vi "Routes.vi"() -> (3 "Routes":T1[](array[typedef]))   [LabVIEW 2024]
doc: "Configure routes"
uses:
  NavigatableView/NavigatableView.lvclass
  Navigator/Route.ctl
  Navigator/Navigator.lvclass
  Pages/Page1/View/View.lvclass
  Pages/Page2/View/View.lvclass
  C:/Users/N Tan/Documents/1-Reuse Modules/Navigator/NavigatableView/NavigatableView.lvclass
  C:/Users/N Tan/Documents/1-Reuse Modules/Navigator/Example/Pages/Page1/View/View.lvclass
  C:/Users/N Tan/Documents/1-Reuse Modules/Navigator/Example/Pages/Page2/View/View.lvclass
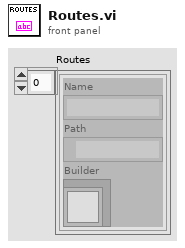
[diagram p1: front panel]
types:
  T1 = typedef "Navigator.lvclass/Route.ctl" = cluster{"Name":string, "Path":path, "Builder":refnum<class "NavigatableView.lvclass">}
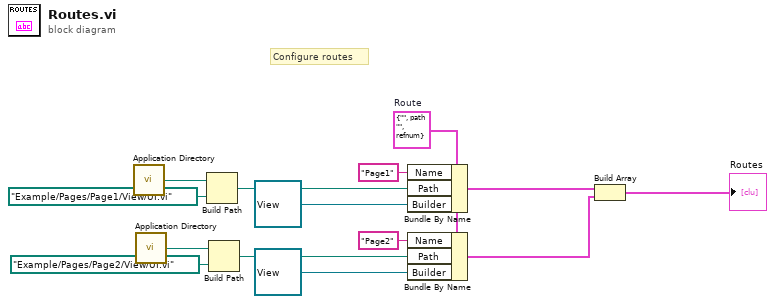
[diagram p0: block diagram]
diagram:
  w10 = T1 {"Name"="", "Path"=path "", "Builder"=refnum}  # Route
  # "Configure routes"
  n1 = call <vilib>:"Application Directory.vi"() -> ("Application Directory"=w8:path)
  n2 = call <vilib>:"Application Directory.vi"() -> ("Application Directory"=w4:path)
  n3 = Build Path(base path=w8, name or relative path=path "Example/Pages/Page1/View/UI.vi") -> (appended path=w6:path)
  n4 = Build Path(base path=w4, name or relative path=path "Example/Pages/Page2/View/UI.vi") -> (appended path=w3:path)
  n5 = Bundle By Name(cluster=w10, "Name"="Page1", "Path"=w6, "Builder"=refnum<class "View.lvclass"> refnum ("Page1.lvlib:View.lvclass")) -> (w13:T1)
  n6 = Bundle By Name(cluster=w10, "Name"="Page2", "Path"=w3, "Builder"=refnum<class "View.lvclass"> refnum ("Page2.lvlib:View.lvclass")) -> (w9:T1)
  n7 = Build Array(w13, w9) -> (→"Routes":T1[])
